vi "PicoScope3000aExampleAWG.vi"() -> ()   [LabVIEW 2009]
uses:
  PS3000a.dll
panel:
  in  "Arbitrary Waveform Settings":T1 {"Index Mode" items=["Single", "Dual", "Quad"]}
  in  "General AWG Settings":T2 {"White Noise/PRBS" items=["Normal", "White Noise", "PRBS"]; "Trigger Source" items=["None", "Scope Trigger", "Aux. In", "Ext. In", "Software Trigger"]; "Trigger Type" items=["Rising", "Falling", "Gate High", "Gate Low"]; "Sweep Type" items=["Up", "Down", "Up-Down", "Down-Up"]; "Wave Type" items=["Sine", "Square", "Triangle", "Ramp Up", "Ramp Down", "DC", "Arbitrary"]}
  in  "Standard Waveform Settings":T3 {"Stop Frequency" min=0.03 max=1000000.0 format="%#_6p"; "Start Frequency" min=0.03 max=1000000.0 format="%#_6p"}
  in  "Stop S/W \nTrigger":bool
  in  "Apply Settings":bool
  in  "Stop VI":bool
  in  "Software \nTrigger":bool
  out "Arbitrary\nWaveform Graph":i16[](graph)
  in  "PS3207A/B device\non non-USB 3.0 Port":bool
  in  "PS34XXA/B devices \nUSB Powered":bool
  # "If Software trigger is selected, press the 'Stop S/W Trigger'\nbutton prior to selecting 'Apply Settings' or 'Stop VI'."
  # "Sweep is disabled when 'Increment' or 'Dwell Time' is set to 0, then 'Start frequency' is used"
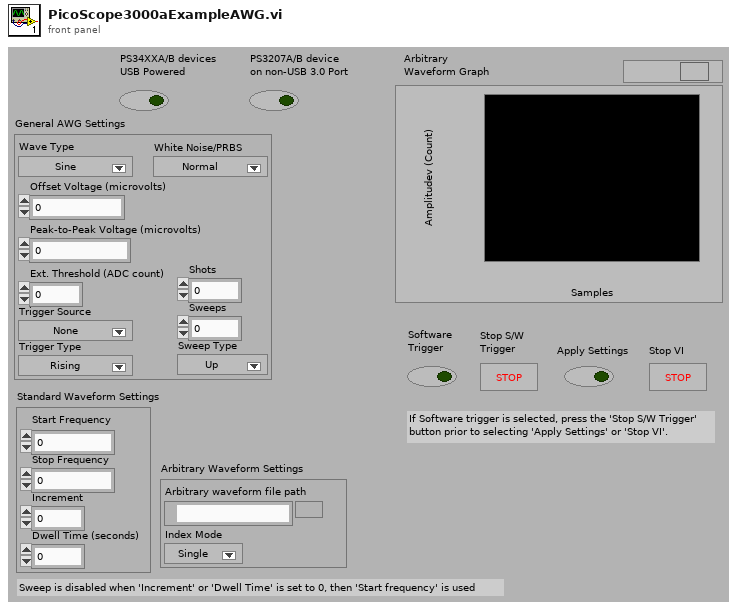
[diagram p1: front panel]
types:
  T1 = cluster{"Arbirary waveform file path":path, "Index Mode":u32}
  T2 = cluster{"Peak-to-Peak Voltage (microvolts)":u32, "Offset Voltage (microvolts)":i32, "Wave Type":i16, "Sweep Type":i32, "Shots":u32, "Sweeps":u32, "Trigger Type":i32, "Trigger Source":i32, "Ext. Threshold (ADC count)":i16, "White Noise/PRBS":u32}
  T3 = cluster{"Start Frequency":dbl, "Stop Frequency":dbl, "Increment":dbl, "Dwell Time (seconds)":dbl}
  T4 = cluster{"Driver Version":string, "USB Version":string, "Hardware":string, "Variant":string, "Batch and Serial":string, "Cal Date":string, "Kernel Version":string, "Digital HW Version":string, "Analogue HW Version":string, "MSO":bool, "Number of channels":i16}
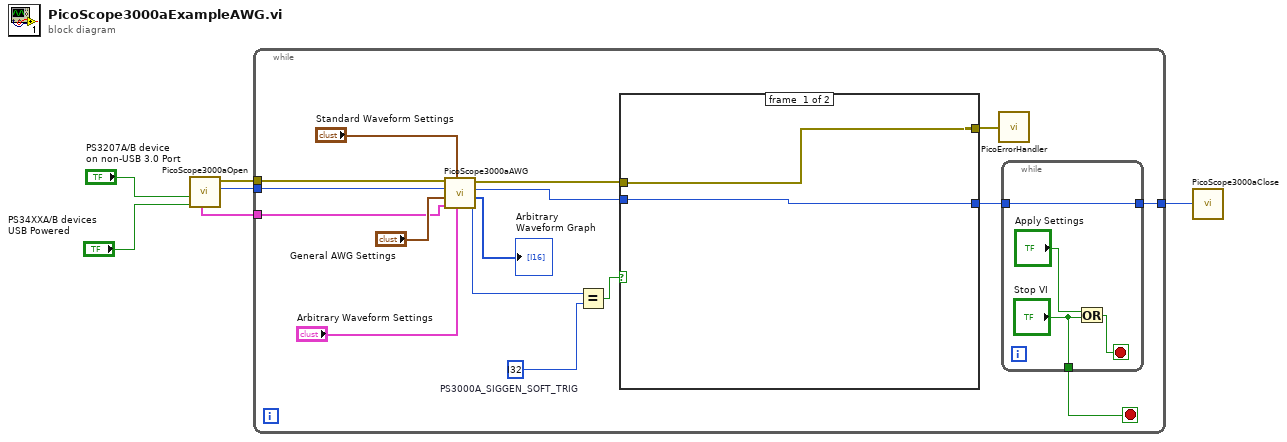
[diagram p0: block diagram]
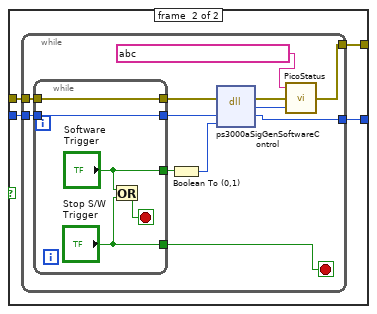
[diagram p2: hidden frame]
diagram:
  n1 = call "PicoScope3000aOpen.vi"("4-channel USB Powered"="PS34XXA/B devices \nUSB Powered", "2-channel USB 3.0 device on non-USB 3.0 Port"="PS3207A/B device\non non-USB 3.0 Port") -> ("handle"=w4:i16, "error out"=w3:errorcluster, "Device Info"=w1:T4)  [unwired: 4 in, 3 out]
  n2 = while {
    tunnel: w4 -> [w21]
    tunnel: w3 -> [w20]
    tunnel: [w14] -> w2
    tunnel: w1 -> [w7]
    stop <- w12 stop-if-true
    w19 = i32 ?  # PS3000A_SIGGEN_SOFT_TRIG
    n3 = call "PicoScope3000aAWG.vi"("Arbitrary Waveform Settings"="Arbitrary Waveform Settings", "Standard Waveform Settings"="Standard Waveform Settings", "Device Info"=w7, "General AWG Settings"="General AWG Settings", "Handle In"=w21, "error in"=w20) -> ("Trigger Source Out"=w15:i32, "Arbitrary\nWaveform Graph"=→"Arbitrary\nWaveform Graph":i16[], "Handle Out"=w16:i16, "error out"=w17:errorcluster)  [unwired: 2 in]
    n4 = Equal?(x=w15, y=w19) -> (x = y?=w18:bool)
    n5 = case shown="True" w18 {
      tunnel: [w28 w29] -> w11
      tunnel: w17 -> [w28 w32]
      tunnel: [w27 w30] -> w13
      tunnel: w16 -> [w27 w31]
      frame #0 {
      }
      frame #1 {
        n6 = while {
          tunnel: w32 -> [w43]
          tunnel: w31 -> [w42]
          tunnel: [w40] -> w30
          tunnel: [w35] -> w29
          stop <- w33 stop-if-true
          n7 = while {
            tunnel: [w49] -> w44
            tunnel: w43 -> [w49]
            tunnel: ["Software \nTrigger"] -> w39
            tunnel: w42 -> [w48]
            tunnel: [w48] -> w41
            tunnel: ["Stop S/W \nTrigger"] -> w33
            stop <- w45 stop-if-true
            n8 = Or(x="Software \nTrigger", y="Stop S/W \nTrigger") -> (x .or. y?=w45:bool)
          }
          n9 = Boolean To (0,1)(Boolean=w39) -> (0, 1=w38:i16)
          n10 = dll-call lib="ps3000a.dll" fn="ps3000aSigGenSoftwareControl"(error in=w44, "handle"=w41, "state"=w38) -> (error out=w36:errorcluster, "PICO_STATUS"=w37:i32, "handle"=w40:i16)  [unwired: 3 in, 1 out]
          n11 = call "PicoStatus.vi"("PICO STATUS"=w37, "error in"=w36, "source"=string ?) -> ("error out"=w35:errorcluster)
        }
      }
    }
    n12 = call "PicoErrorHandler.vi"("error in"=w11) -> ()  [unwired: 1 out]
    n13 = while {
      tunnel: ["Stop VI"] -> w12
      tunnel: [w26] -> w14
      tunnel: w13 -> [w26]
      stop <- w25 stop-if-true
      n14 = Or(x="Apply Settings", y="Stop VI") -> (x .or. y?=w25:bool)
    }
  }
  n15 = call "PicoScope3000aClose.vi"("handle"=w2) -> ()
